vi "Update Plot Legends.vi"(7 "Update Config (F)":bool, 8 "error in (no error)":errorcluster, 11 "HistorianCharting in":refnum<class "HistorianCharting.lvclass">) -> (0 "error out":errorcluster, 3 "HistorianCharting out":refnum<class "HistorianCharting.lvclass">)   [LabVIEW 2020, in "VolatusGUIElements.lvlib" / "HistorianCharting.lvclass"]
uses:
  HistorianCharting.lvclass
  HistorianCharting.lvclass/HistorianCharting.ctl
  VolatusGUI/Historian Charting Manager/Scale.ctl
  Volatus/VolatusAPI/VolatusAPI.lvclass/VolatusAPI.ctl
  lv-vecto/Vecto/Channel DBL/Channel DBL.lvclass/Channel DBL.ctl
  lv-vecto/Vecto/ChannelService/Lookup Double Channel.vi
  lv-vecto/Vecto/Group DBL/Value by Index.vi
  VolatusGUI/Historian Charting Manager/Historian Charting Manager.lvclass
  lv-vecto/Vecto/Channel DBL/Channel DBL.lvclass
  Volatus/VolatusAPI/VolatusAPI.lvclass
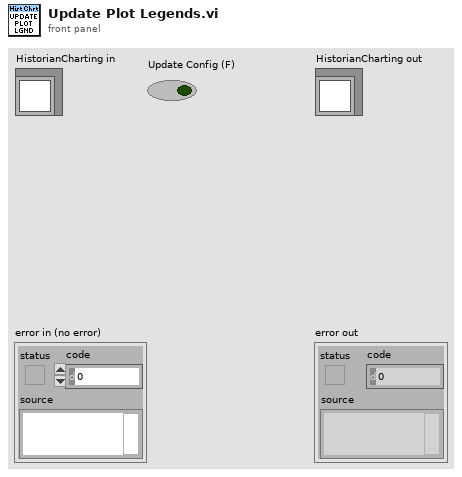
[diagram p1: front panel]
types:
  T1 = typedef "VolatusGUI.lvlib/Historian Charting Manager.lvclass/Plot Config.ctl" = cluster{"Channel":string, "Visible":bool, "Color":u32, "Scale":T2}
  T2 = typedef "VolatusGUI.lvlib/Historian Charting Manager.lvclass/Scale.ctl" = enum16{"Left", "Right"}
  T3 = cluster{"Channel":string, "Value":dbl, "Color":u32, "Scale":bool, "Visible":bool}
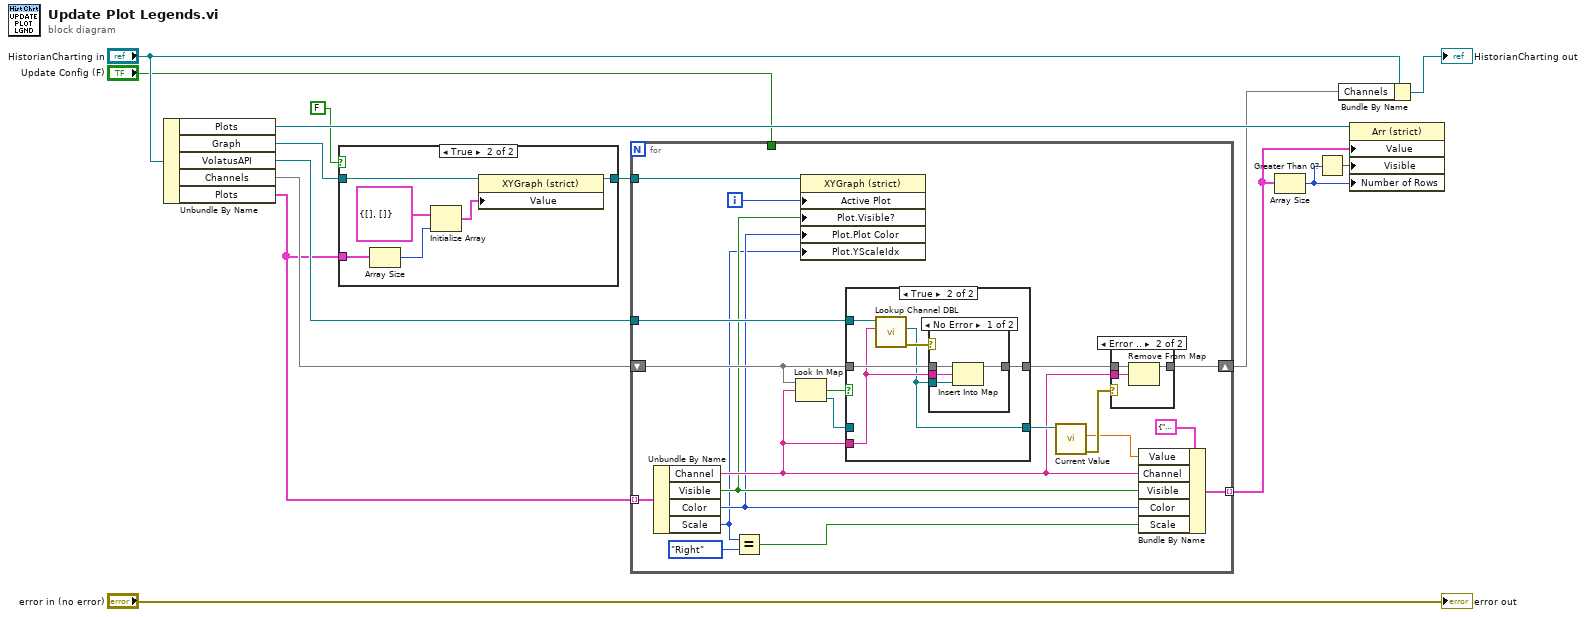
[diagram p0: block diagram]
diagram:
  n1 = Unbundle By Name("HistorianCharting in") -> ("Plots"=w13:refnum<vi>, "Graph"=w5:refnum<vi>, "VolatusAPI"=w11:refnum<class "VolatusAPI.lvclass">, "Channels"=w12:map{string, refnum<class "Channel DBL.lvclass">}, "Plots"=w4:T1[])
  n2 = case shown="True" FALSE {
    tunnel: w5 -> [w16 w22]
    tunnel: w4 -> [_ w21]
    tunnel: [w16 w19] -> w3
    frame False {
    }
    frame True {
      n3 = Array Size(array=w21) -> (size(s)=w17:i32)
      n4 = Initialize Array(cluster{dbl[], dbl[]} {[], []}, w17) -> (w18:cluster{dbl[], dbl[]}[])
      n5 = property class="XYGraph (strict)"(reference=w22, "Value"=w18) -> (reference out=w19:refnum<vi>)  [unwired: 1 in, 1 out]
    }
  }
  n6 = for {
    tunnel: w4 -> [w41] mode=indexing
    tunnel: [w37] -> w8 mode=indexing
    shift-right: [w29] -> w9
    shift-left: w12 -> [w32]
    tunnel: w11 -> [w31]
    tunnel: w3 -> [w27]
    tunnel: "Update Config (F)" -> [_]
    i -> [w26]
    n7 = Unbundle By Name(w41) -> ("Channel"=w28:string, "Visible"=w25:bool, "Color"=w24:u32, "Scale"=w23:T2)
    n8 = Equal?(x=w23, y=Scale."Right") -> (x = y?=w38:bool)
    n9 = Look In Map(map=w32, key=w28) -> (key not found?=w36:bool, value=w35:refnum<class "Channel DBL.lvclass">)  [unwired: 1 in]
    n10 = property class="XYGraph (strict)"(reference=w27, "Active Plot"=w26, "Plot.Visible?"=w25, "Plot.Plot Color"=w24, "Plot.YScaleIdx"=w23) -> ()  [unwired: 1 in, 2 out]
    n11 = case shown="True" w36 {
      tunnel: w35 -> [w48 _]
      tunnel: [w48 w50] -> w34
      tunnel: w32 -> [w47 w52]
      tunnel: w28 -> [_ w51]
      tunnel: w31 -> [_ w53]
      tunnel: [w47 w49] -> w30
      frame False {
      }
      frame True {
        n12 = call "Lookup Channel DBL.vi"("Name"=w51, "VolatusAPI in"=w53) -> ("error out"=w54:errorcluster, "Channel DBL"=w50:refnum<class "Channel DBL.lvclass">)  [unwired: 7 in, 1 out]
        n13 = case shown="No Error" w54 {
          tunnel: w52 -> [w58 w59]
          tunnel: w51 -> [w57 _]
          tunnel: w50 -> [w56 _]
          tunnel: [w55 w59] -> w49
          frame No Error {
            n14 = Insert Into Map(map in=w58, key=w57, value=w56) -> (map out=w55:map{string, refnum<class "Channel DBL.lvclass">})  [unwired: 2 out]
          }
          frame Error {
          }
        }
      }
    }
    n15 = call "Current Value.vi"("Channel in"=w34) -> ("error out"=w42:errorcluster, "Scaled"=w33:dbl)  [unwired: 6 in, 3 out]
    n16 = case shown="Error .." w42 {
      tunnel: w30 -> [w43 w46]
      tunnel: [w43 w45] -> w29
      tunnel: w28 -> [_ w44]
      frame No Error {
      }
      frame Error {
        n17 = Remove From Map(10:w44, 11:w46) -> (3:w45:map{string, refnum<class "Channel DBL.lvclass">})  [unwired: 2 out]
      }
    }
    n18 = Bundle By Name(cluster=T3 {"Channel"="", "Value"=0.0, "Color"=16777215, "Scale"=FALSE, "Visible"=FALSE} ("Plot"), "Value"=w33, "Channel"=w28, "Visible"=w25, "Color"=w24, "Scale"=w38) -> (w37:T3)
  }
  n19 = Array Size(array=w8) -> (size(s)=w7:i32)
  n20 = Greater Than 0?(x=w7) -> (x > 0?=w6:bool)
  n21 = Bundle By Name(cluster="HistorianCharting in", "Channels"=w9) -> (→"HistorianCharting out":refnum<class "HistorianCharting.lvclass">)
  n22 = property class="Arr (strict)"(reference=w13, "Value"=w8, "Visible"=w6, "Number of Rows"=w7) -> ()  [unwired: 1 in, 2 out]
  "error out" <- "error in (no error)"
